vi "Convert Inches to Sensor Position.vi"(11 "Cascade Setpoints Config in":T2) -> (3 "Cluster":cluster{cluster{"Preset Name":T1, dbl}[]})   [LabVIEW 2027]
uses:
  Cascade Positions.ctl
  <vilib>/Rock Robotics/Network Tables/NT Read Numeric Array.vi
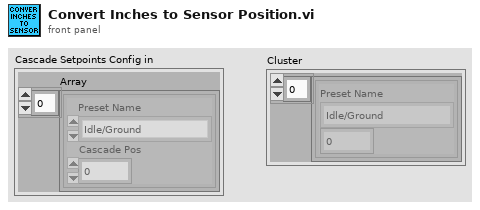
[diagram p1: front panel]
types:
  T1 = typedef "Cascade Positions.ctl" = enum16{"Idle/Ground", "Raised L1", "L2", "L2 Tip", "L3", "L3 Tip", "Feeder", "\"Default\""}
  T2 = cluster{"Array":cluster{"Preset Name":T1, "Cascade Pos":dbl}[]}
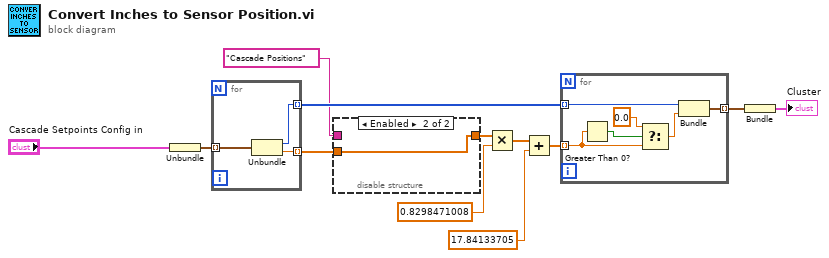
[diagram p0: block diagram]
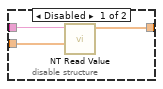
[diagram p2: hidden frame]
diagram:
  n1 = Unbundle("Cascade Setpoints Config in") -> ("Array"=w2:cluster{"Preset Name":T1, "Cascade Pos":dbl}[])
  n2 = for {
    tunnel: w2 -> [w15] mode=indexing
    tunnel: [w14] -> w3 mode=indexing
    tunnel: [w13] -> w9 mode=indexing
    n3 = Unbundle(w15) -> ("Preset Name"=w13:T1, "Cascade Pos"=w14:dbl)
  }
  n4 = disable-structure shown="Enabled" {
    disable-tunnel: [w18 w19] -> w5
    disable-tunnel: "Cascade Positions" ("name") -> [w17 _]
    disable-tunnel: w3 -> [w16 w19]
    frame Disabled {
      n5 = call-poly <vilib>:"NT Read Value.vi"("default value"=w16, "name"=w17) -> ("value"=w18:dbl[])  [unwired: 7 in, 2 out]
    }
    frame Enabled {
    }
  }
  n6 = Multiply(x=w5, y=0.8298471008) -> (x*y=w7:dbl[])
  n7 = Add(x=w7, y=17.84133705) -> (x+y=w10:dbl[])
  n8 = for {
    tunnel: w9 -> [w25] mode=indexing
    tunnel: w10 -> [w21] mode=indexing
    tunnel: [w24] -> w11 mode=indexing
    n9 = Greater Than 0?(x=w21) -> (x > 0?=w23:bool)
    n10 = Select(t=0.0, s=w23, f=w21) -> (s? t:f=w20:dbl)
    n11 = Bundle("Preset Name"=w25, "t"=w20) -> (w24:cluster{"Preset Name":T1, "t":dbl})  [unwired: 1 in]
  }
  n12 = Bundle(w11) -> (→"Cluster":cluster{cluster{"Preset Name":T1, "t":dbl}[]})  [unwired: 1 in]
